vi "AO 薄膜(子VI) - PS2.vi"(9 "电压":dbl caption="数据" format="%0.2f", 10 "VISA资源名称":refnum<visa-resource-name>) -> (2 "返回信息":u8[](array[numeric]))   [LabVIEW 2026, in "UI-压力.lvlib" / "Acquisition.lvlib"]
uses:
  Acquisition.lvlib
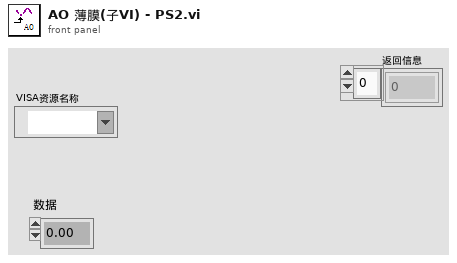
[diagram p1: front panel]
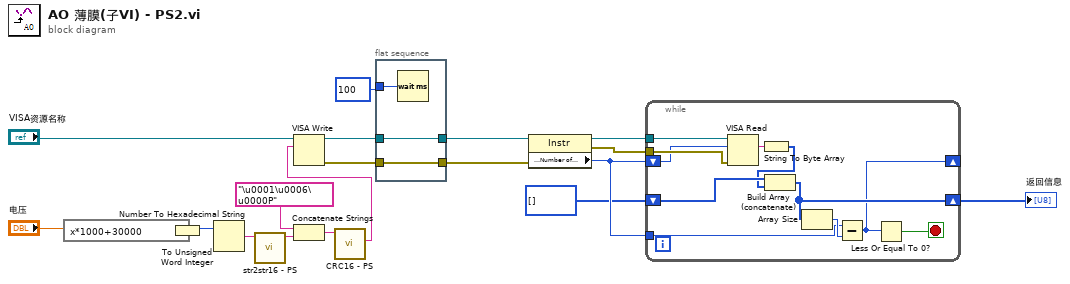
[diagram p0: block diagram]
diagram:
  n1 = expression code="x*1000+30000"("电压") -> (w8:dbl)
  n2 = To Unsigned Word Integer(number=w8) -> (unsigned 16bit integer=w2:u16)
  n3 = Number To Hexadecimal String(2:w2) -> (0:w6:string)  [unwired: 1 in]
  n4 = call "str2str16 - PS.vi"("字符串"=w6) -> ("string"=w5:string)  [unwired: 10 in]
  n5 = Concatenate Strings("\u0001\u0006\u0000P" ("字符串"), w5) -> (w4:string)
  n6 = call "CRC16 - PS.vi"("要校验的字符串（十六进制显示）"=w4) -> ("连接的字符串(16进制)"=w1:string)  [unwired: 9 in, 1 out]
  n7 = VISA Write(VISA resource name="VISA资源名称", write buffer=w1) -> (VISA resource name out=w15:refnum<visa-resource-name>, error out=w13:errorcluster)  [unwired: 1 in, 1 out]
  n8 = flat-sequence {
    tunnel: w13 -> [w21]
    tunnel: [w21] -> w14
    tunnel: w15 -> [w20]
    tunnel: [w20] -> w16
    tunnel: u32 100 ("读取前延时(ms)") -> [w22]
    frame #0 {
      n9 = Wait (ms)(milliseconds to wait=w22) -> ()  [unwired: 1 out]
    }
  }
  n10 = property class="Instr"(reference=w16, error in=w14) -> (reference out=w17:refnum<visa-resource-name>, error out=w18:errorcluster, "Serial Settings:Number of Bytes at Serial Port"=w19:u32)
  n11 = while {
    tunnel: w17 -> [w31]
    tunnel: w18 -> [w30]
    shift-right: [w33] -> w7
    shift-left: u8[] [] ("unsigned byte array") -> [w32]
    tunnel: w19 -> [w25]
    shift-right: [w23] -> _
    shift-left: w19 -> [w29]
    stop <- w24 stop-if-true
    n12 = VISA Read(VISA resource name=w31, byte count=w29, error in (no error)=w30) -> (read buffer=w28:string)  [unwired: 3 out]
    n13 = String To Byte Array(string=w28) -> (unsigned byte array=w27:u8[])
    n14 = Build Array (concatenate)(w32, w27) -> (w33:u8[])
    n15 = Array Size(array=w33) -> (size(s)=w26:i32)
    n16 = Subtract(x=w25, y=w26) -> (x-y=w23:u32)
    n17 = Less Or Equal To 0?(x=w23) -> (x <= 0?=w24:bool)
  }
  "返回信息" <- w7
